vi "ActiveObject_QueueQueue_ProcessRepository_Native.vi"(0 "reference in":refnum<class>, 1 "Action(ReadRepository)":T1(ring), 5 "Error In":errorcluster) -> (9 "ProcessViRef":refnum<vi>, 11 "ProcessSyncQueue":refnum<queue>, 13 "FromProcessQueue":refnum<queue>, 14 "reference out":refnum<class>, 15 "ToProcessQueue":refnum<queue>, 17 "ProcessAlreadyStarted":bool, 19 "Error Out":errorcluster)   [LabVIEW 2020]
uses:
  ActiveObject_QueueQueue_Process.ctl
panel:
  # "Use this indicator for sending messages to the Process VI"
  # "These indicators are used by the process VIs"
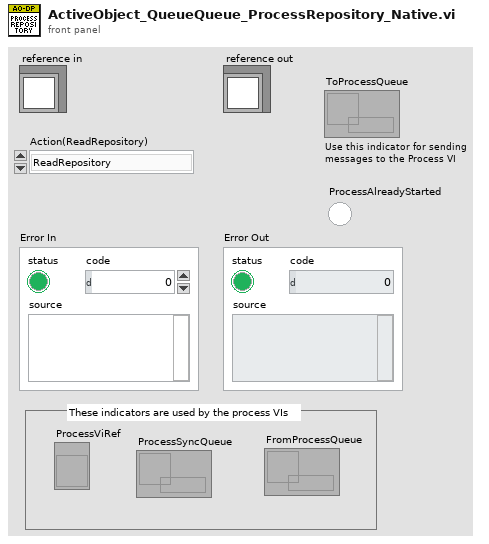
[diagram p1: front panel]
types:
  T1 = enum16{"ReadRepository", "CreateNew", "CreateOrLookUpExisting", "ReadRepositoryAndDestroy"}
  T2 = typedef "ActiveObject_QueueQueue_Process.ctl" = cluster{"ToProcessQueue":refnum<queue>, "FromProcessQueue":refnum<queue>, "ProcessSyncQueue":refnum<queue>, "ProcessViRef":refnum<vi>}
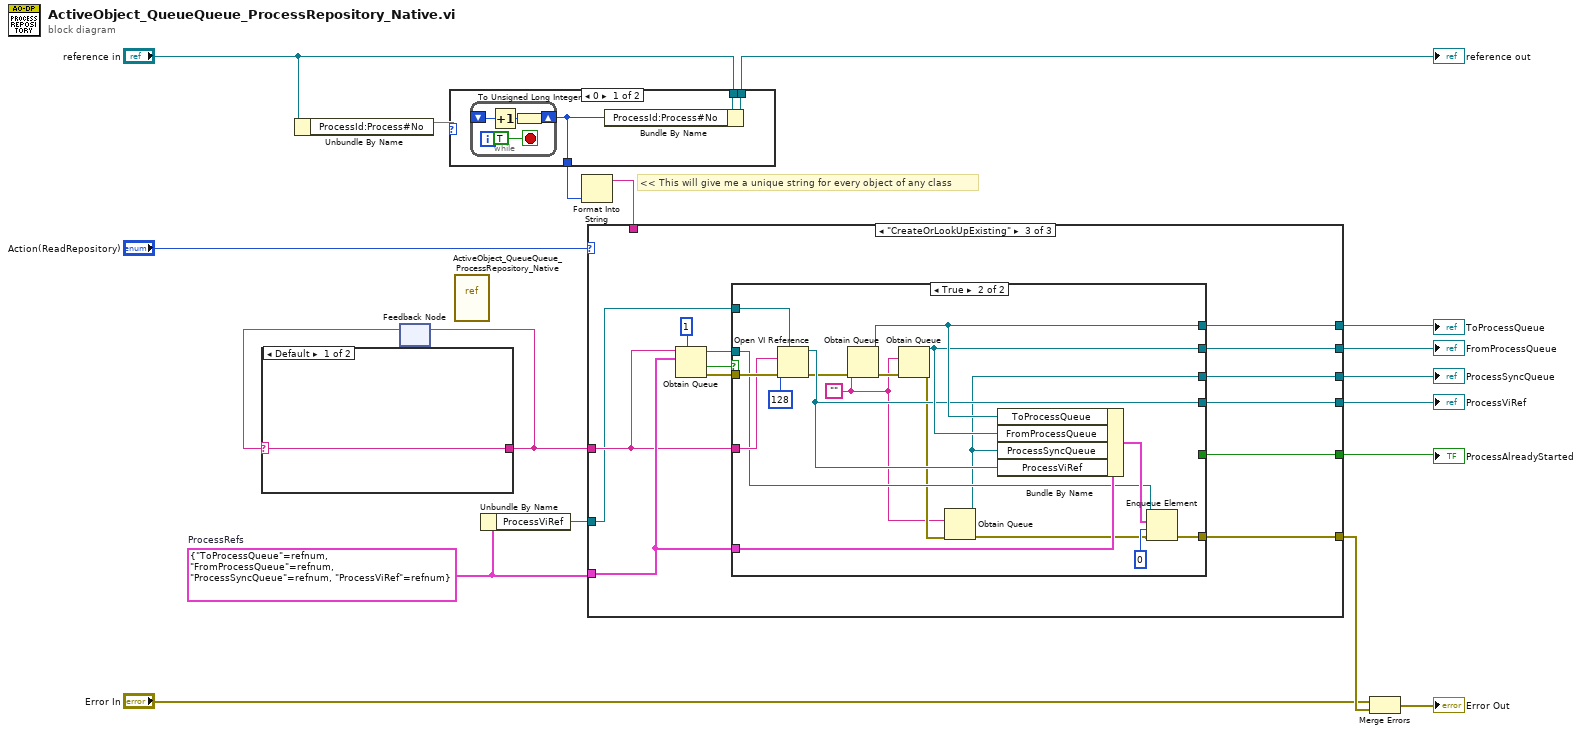
[diagram p0: block diagram]
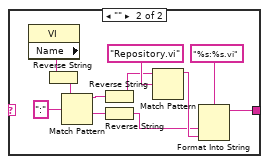
[diagram p2: hidden frame]
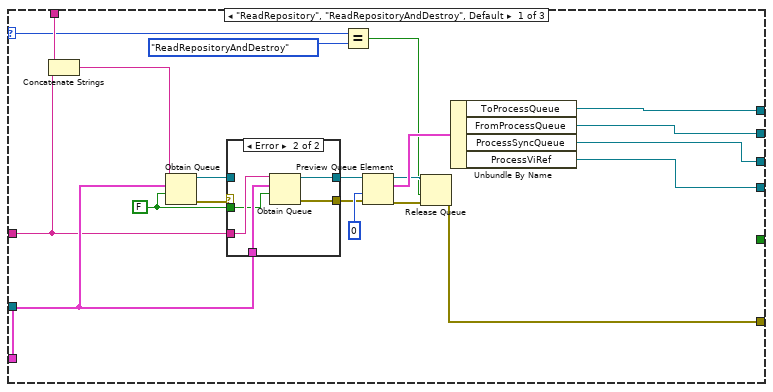
[diagram p4: hidden frame]
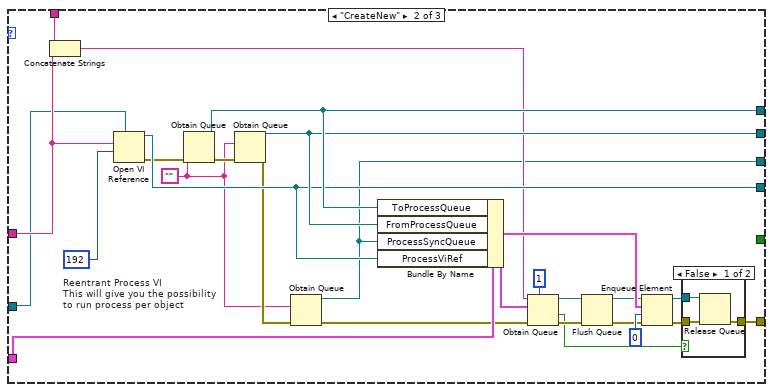
[diagram p6: hidden frame]
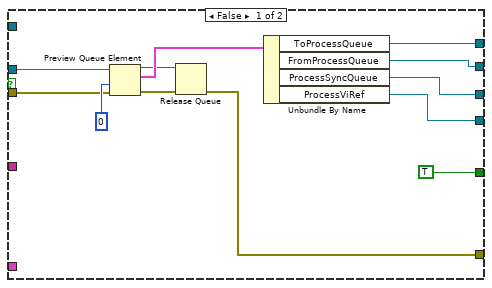
[diagram p8: hidden frame]
diagram:
  w4 = T2 {"ToProcessQueue"=refnum, "FromProcessQueue"=refnum, "ProcessSyncQueue"=refnum, "ProcessViRef"=refnum}  # ProcessRefs
  # "<< This will give me a unique string for every object of any class"
  n1 = Unbundle By Name("reference in") -> ("ProcessId:Process#No"=w8)
  n2 = feedback #1() -> (w1:string)  [unwired: 1 in]
  n3 = case shown="Default" w1 {
    selector: w1 -> [w19 _]
    tunnel: [w19 w20] -> w2
    frame Default {
    }
    frame "" {
      n4 = property class="VI"() -> ("Name"=w22:string)  [unwired: 2 in, 2 out]
      n5 = Reverse String(1:w22) -> (0:w23:string)
      n6 = Match Pattern(string=w23, regular expression=":") -> (before substring=w27:string, after substring=w24:string)  [unwired: 1 in, 2 out]
      n7 = Reverse String(1:w27) -> (0:w28:string)
      n8 = Reverse String(1:w24) -> (0:w26:string)
      n9 = Match Pattern(string=w28, regular expression="Repository.vi") -> (before substring=w30:string)  [unwired: 1 in, 3 out]
      n10 = Format Into String(format string="%s:%s.vi", w26, w30) -> (resulting string=w20:string)  [unwired: 2 in, 1 out]
    }
  }
  n11 = feedback-in #1(w2) -> ()
  n12 = case shown="0" w8 {
    selector: w8 -> [_ w39]
    tunnel: [w31 w39] -> w9
    tunnel: "reference in" -> [w33 w38]
    tunnel: [w32 w38] -> w6
    frame 0 {
      n13 = while {
        shift-right: [w34] -> w31
        shift-left: _ -> [w36]
        stop <- TRUE stop-if-true
        n14 = Increment(x=w36) -> (x+1=w35:u32)
        n15 = To Unsigned Long Integer(number=w35) -> (unsigned 32bit integer=w34:u32)
      }
      n16 = Bundle By Name(cluster=w33, "ProcessId:Process#No"=w31) -> (w32:refnum<class>)
    }
    frame Default {
    }
  }
  "reference out" <- w6
  n17 = vi-ref "ActiveObject_QueueQueue_ProcessRepository_Native.vi"() -> ()  [unwired: 1 out]
  n18 = Unbundle By Name(w4) -> ("ProcessViRef"=w3:refnum<vi>)
  n19 = Format Into String(w9) -> (resulting string=w5:string)  [unwired: 3 in, 1 out]
  n20 = case shown="\"CreateOrLookUpExisting\"" "Action(ReadRepository)" {
    selector: "Action(ReadRepository)" -> [w42 _ _]
    tunnel: [w55 w76 w108] -> w17
    tunnel: [w57 w93 w110] -> w15
    tunnel: [w56 w92 w109] -> w16
    tunnel: [w58 w91 w107] -> w14
    tunnel: w4 -> [w50 w83 w103]
    tunnel: w5 -> [w48 w82 _]
    tunnel: [w43 w70 w106] -> w12
    tunnel: w2 -> [w47 w80 w99]
    tunnel: [_ _ w101] -> w11
    tunnel: w3 -> [_ w68 w98]
    frame "ReadRepository", "ReadRepositoryAndDestroy", Default {
      w49 = FALSE ("create if not found? (T)")
      n21 = Concatenate Strings(w48, w47) -> (w46:string)
      n22 = Obtain Queue(name (unnamed)=w46, element data type=w50, create if not found? (T)=w49) -> (queue out=w52:refnum<queue>, error out=w54:errorcluster)  [unwired: 2 in, 1 out]
      n23 = case shown="Error" w54 {
        selector: w54 -> [w62 _]
        tunnel: [w62 w64] -> w53
        tunnel: w52 -> [w61 _]
        tunnel: [w61 w65] -> w51
        tunnel: w50 -> [_ w67]
        tunnel: w47 -> [_ w66]
        tunnel: w49 -> [_ w63]
        frame No Error {
        }
        frame Error {
          n24 = Obtain Queue(name (unnamed)=w66, element data type=w67, create if not found? (T)=w63) -> (queue out=w65:refnum<queue>, error out=w64:errorcluster)  [unwired: 2 in, 1 out]
        }
      }
      n25 = Equal?(x=w42, y=T1."ReadRepositoryAndDestroy") -> (x = y?=w41:bool)
      n26 = Preview Queue Element(queue=w51, timeout in ms (-1)=0, error in (no error)=w53) -> (queue out=w45:refnum<queue>, element=w59:T2, error out=w44:errorcluster)  [unwired: 1 out]
      n27 = Release Queue(queue=w45, force destroy? (F)=w41, error in (no error)=w44) -> (error out=w43:errorcluster)  [unwired: 2 out]
      n28 = Unbundle By Name(w59) -> ("ToProcessQueue"=w57:refnum<queue>, "FromProcessQueue"=w56:refnum<queue>, "ProcessSyncQueue"=w55:refnum<queue>, "ProcessViRef"=w58:refnum<vi>)
    }
    frame "CreateNew" {
      w88 = 192  # Reentrant Process VI This will give you the possibility to run process per object
      w77 = ""
      n29 = Concatenate Strings(w82, w80) -> (w81:string)
      n30 = Open VI Reference(type specifier VI Refnum (for type only)=w68, vi path=w80, options=w88) -> (vi reference=w91:refnum<vi>, error out=w89:errorcluster)  [unwired: 3 in]
      n31 = Obtain Queue(element data type=w77, error in (no error)=w89) -> (queue out=w93:refnum<queue>, error out=w90:errorcluster)  [unwired: 3 in, 1 out]
      n32 = Obtain Queue(element data type=w77, error in (no error)=w90) -> (queue out=w92:refnum<queue>, error out=w79:errorcluster)  [unwired: 3 in, 1 out]
      n33 = Obtain Queue(element data type=w77, error in (no error)=w79) -> (queue out=w76:refnum<queue>, error out=w78:errorcluster)  [unwired: 3 in, 1 out]
      n34 = Bundle By Name(cluster=w83, "ToProcessQueue"=w93, "FromProcessQueue"=w92, "ProcessSyncQueue"=w76, "ProcessViRef"=w91) -> (w86:T2)
      n35 = Obtain Queue(max queue size (-1, unlimited)=1, name (unnamed)=w81, element data type=w86, error in (no error)=w78) -> (queue out=w87:refnum<queue>, created new?=w69:bool, error out=w74:errorcluster)  [unwired: 1 in]
      n36 = Flush Queue(queue=w87, error in (no error)=w74) -> (queue out=w75:refnum<queue>, error out=w73:errorcluster)  [unwired: 1 out]
      n37 = Enqueue Element(queue=w75, element=w86, timeout in ms (-1)=0, error in (no error)=w73) -> (queue out=w71:refnum<queue>, error out=w72:errorcluster)  [unwired: 1 out]
      n38 = case shown="False" w69 {
        tunnel: w72 -> [w96 w97]
        tunnel: w71 -> [w95 _]
        tunnel: [w94 w97] -> w70
        frame False {
          n39 = Release Queue(queue=w95, error in (no error)=w96) -> (error out=w94:errorcluster)  [unwired: 1 in, 2 out]
        }
        frame True {
        }
      }
    }
    frame "CreateOrLookUpExisting" {
      n40 = Obtain Queue(max queue size (-1, unlimited)=1, name (unnamed)=w99, element data type=w103) -> (queue out=w104:refnum<queue>, created new?=w105:bool, error out=w102:errorcluster)  [unwired: 2 in]
      n41 = case shown="True" w105 {
        tunnel: [w122 w140] -> w110
        tunnel: [w121 w139] -> w109
        tunnel: [w120 w125] -> w108
        tunnel: [w119 w138] -> w107
        tunnel: [w112 w137] -> w106
        tunnel: w103 -> [_ w136]
        tunnel: w102 -> [w116 w131]
        tunnel: w99 -> [_ w130]
        tunnel: w104 -> [w117 w129]
        tunnel: [TRUE _] -> w101
        tunnel: w98 -> [_ w124]
        frame False {
          n42 = Preview Queue Element(queue=w117, timeout in ms (-1)=0, error in (no error)=w116) -> (queue out=w111:refnum<queue>, element=w115:T2, error out=w113:errorcluster)  [unwired: 1 out]
          n43 = Release Queue(queue=w111, error in (no error)=w113) -> (error out=w112:errorcluster)  [unwired: 1 in, 2 out]
          n44 = Unbundle By Name(w115) -> ("ToProcessQueue"=w122:refnum<queue>, "FromProcessQueue"=w121:refnum<queue>, "ProcessSyncQueue"=w120:refnum<queue>, "ProcessViRef"=w119:refnum<vi>)
        }
        frame True {
          w126 = ""
          n45 = Open VI Reference(type specifier VI Refnum (for type only)=w124, vi path=w130, options=128, error in (no error)=w131) -> (vi reference=w138:refnum<vi>, error out=w134:errorcluster)  [unwired: 2 in]
          n46 = Obtain Queue(element data type=w126, error in (no error)=w134) -> (queue out=w140:refnum<queue>, error out=w135:errorcluster)  [unwired: 3 in, 1 out]
          n47 = Obtain Queue(element data type=w126, error in (no error)=w135) -> (queue out=w139:refnum<queue>, error out=w128:errorcluster)  [unwired: 3 in, 1 out]
          n48 = Obtain Queue(element data type=w126, error in (no error)=w128) -> (queue out=w125:refnum<queue>, error out=w127:errorcluster)  [unwired: 3 in, 1 out]
          n49 = Bundle By Name(cluster=w136, "ToProcessQueue"=w140, "FromProcessQueue"=w139, "ProcessSyncQueue"=w125, "ProcessViRef"=w138) -> (w133:T2)
          n50 = Enqueue Element(queue=w129, element=w133, timeout in ms (-1)=0, error in (no error)=w127) -> (error out=w137:errorcluster)  [unwired: 2 out]
        }
      }
    }
  }
  "ProcessSyncQueue" <- w17
  "ToProcessQueue" <- w15
  "FromProcessQueue" <- w16
  "ProcessViRef" <- w14
  "ProcessAlreadyStarted" <- w11
  n51 = Merge Errors("Error In", w12) -> (→"Error Out":errorcluster)
